vi "Create.vi"(6 "Label Names":string[](array[string]), 7 "Registry Name":string="_default_registry", 8 "error in (no error)":errorcluster, 9 "Auto-register?":bool=TRUE, 10 "Description":string, 11 "Metric Name":string) -> (0 "error out":errorcluster, 3 "Gauge Ref":refnum<data-value>)   [LabVIEW 2020, in "Metrics.lvlib" / "Gauge.lvclass"]
doc: "Creates a gauge metric. A gauge can go up and down, or be set to an arbitrary value."
uses:
  Gauge.lvclass
  C:/Github-locals/PromVIEW/src/metrics/metric/Metric.lvclass
  metric/Metric.lvclass/Metric.ctl
  metric/Write Name.vi
  metric/Write Description.vi
  metric/Write Label Names.vi
  metric/Validate Name.vi
  registry/session/Registry Session.lvclass
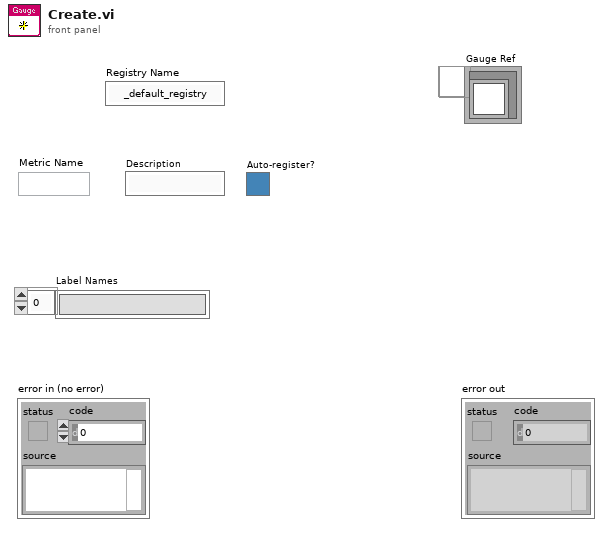
[diagram p1: front panel]
types:
  T1 = typedef "Registry.lvlib/Registry Session.lvclass/Session Handle.ctl" = refnum<data-value>
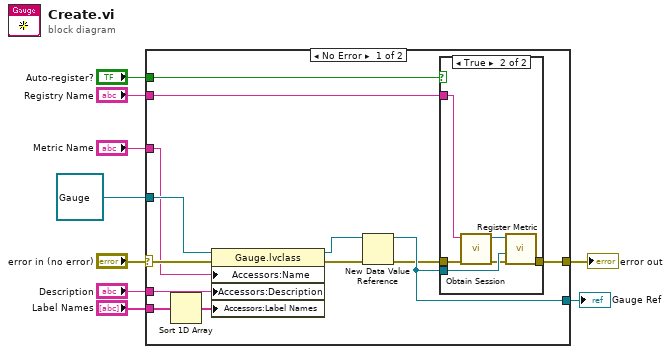
[diagram p0: block diagram]
diagram:
  n1 = case shown="No Error" "error in (no error)" {
    selector: "error in (no error)" -> [w15 w30]
    tunnel: [w19 w30] -> w8
    tunnel: "Metric Name" -> [w13 _]
    tunnel: "Label Names" -> [w14 _]
    tunnel: "Description" -> [w21 _]
    tunnel: refnum<class "Gauge.lvclass"> refnum ("Metrics.lvlib:Gauge.lvclass") -> [w22 _]
    tunnel: [w18 _] -> w1
    tunnel: "Registry Name" -> [w20 _]
    tunnel: "Auto-register?" -> [w16 _]
    frame No Error {
      n2 = Sort 1D Array(array=w14) -> (sorted array=w10:string[])
      n3 = property class="Gauge.lvclass"(reference=w22, error in=w15, "Accessors:Name"=w13, "Accessors:Description"=w21, "Accessors:Label Names"=w10) -> (reference out=w12:refnum<class "Gauge.lvclass">, error out=w11:errorcluster)
      n4 = New Data Value Reference(data value=w12, error in=w11) -> (data value reference=w18:refnum<data-value>, error out=w17:errorcluster)
      n5 = case shown="True" w16 {
        tunnel: w20 -> [_ w29]
        tunnel: [w23 w28] -> w19
        tunnel: w18 -> [_ w27]
        tunnel: w17 -> [w23 w25]
        frame False {
        }
        frame True {
          n6 = call "Obtain Session.vi"("error in (no error)"=w25, "Session  Name ()"=w29) -> ("error out"=w24:errorcluster, "Session Handle"=w26:T1)  [unwired: 8 in]
          n7 = call "Register Metric.vi"("error in (no error)"=w24, "New Metric"=w27, "Session Handle in"=w26) -> ("error out"=w28:errorcluster)  [unwired: 7 in, 1 out]
        }
      }
    }
    frame Error {
    }
  }
  "error out" <- w8
  "Gauge Ref" <- w1
